vi "SMR_LabVIEW_V9.1.vi"() -> ()   [LabVIEW 2025]
uses:
  Control 1.ctl
  <vilib>/DAQmx/write.llb/DAQmx Write (Analog DBL 1Chan 1Samp).vi
  <vilib>/DAQmx/read.llb/DAQmx Read (Analog 1D DBL NChan 1Samp).vi
  <vilib>/DAQmx/read.llb/DAQmx Read (Analog 2D DBL NChan NSamp).vi
  <vilib>/Analysis/baseanly.llb/Mean (DBL).vi
  <vilib>/DAQmx/create/channels.llb/DAQmx Create Channel (AI-Temperature-Thermocouple).vi
  <vilib>/DAQmx/create/channels.llb/DAQmx Create Channel (AI-Voltage-Basic).vi
  <vilib>/DAQmx/create/channels.llb/DAQmx Create Channel (AO-Voltage-Basic).vi
  <vilib>/DAQmx/miscellaneous.llb/DAQmx Fill In Error Info.vi
  <vilib>/DAQmx/configure/timing.llb/DAQmx Timing (Sample Clock).vi
  <vilib>/DAQmx/create/channels.llb/DAQmx Create Channel (AO-Current-Basic).vi
  <vilib>/addons/control/pid/pid.llb/PID (DBL).vi
  <vilib>/measure/maspectr.llb/FFT Power Spectrum and PSD for 1 Chan.vi
  <vilib>/measure/matone.llb/Extract Single Tone Information 1 Chan.vi
  <vilib>/addons/control/pid/NI_PID_pid.lvlib
  <vilib>/Analysis/NI_AALBase.lvlib
  <vilib>/ptbypt/NI_PtbyPt.lvlib
  <vilib>/measure/NI_MAPro.lvlib
panel:
  in  "R Burden (Ohm)":T1=220.0 min=220.0 max=220.0
  out "PSU Command (mA)":dbl
  in  "PSU Power Setpoint (W)":dbl
  in  "Manual PSU Command (0-8.5)":dbl min=0.0 max=8.5
  in  "PSU: Manual/ PID (on)":bool
  out "Room Temp (deg C)":dbl
  out "HW Valve Command (V)":dbl
  in  "HX Flow Setpoint (GPM)":dbl
  in  "Manual HW Valve Command (V)":dbl min=0.0 max=10.0
  in  "HW Valve: Manual / PID (on)":bool
  in  "PID gains for HW Valve":T2={"proportional gain (Kc)"=1.0, "integral time (Ti, min)"=0.01, "derivative time (Td, min)"=0.0} {"derivative time (Td, min)" format="%.3f"; "integral time (Ti, min)" format="%.3f"; "proportional gain (Kc)" format="%.3f"}
  out "Rod Power (W)":dbl
  out "Current Through Rod (A)":dbl
  out "Time in Steady State (s)":dbl
  in  "Steady-State Dwell (s)":dbl
  out "Main Loop Flow (GPM)":dbl
  out "FM Amplitude":dbl
  out "FM Frequency":dbl
  out "Spectrum":cluster{"f0":dbl, "df":dbl, "magnitude":dbl[]}(graph)
  out "Raw Signal":waveform(dbl)(graph)
  out "Smoothed HX Flow (GPM)":dbl
  out "Flow History":dbl(graph)
  out "HX Flow (GPM)":dbl
  out "Voltage Across Rod (V)":dbl format="%0.2f"
  out "Current Run Folder":path
  in  "Log Root Folder":path=path "C:/Users/LocalUser/Documents/GitHub/thermal-loop/resources/v0.1.1/data/001"
  out "Raw NI9201 \nVoltage Display":T3
  in  "Loop Period (ms)":dbl=1000.0
  in  "Stop":bool
  out "Auto Steady State Threshold (deg C/min)":dbl
  out "Max dT/dt (deg C/min)":dbl
  out "Temp Change Rate (deg C/min)":dbl
  out "5-Min Baseline Complete":bool
  out "Rate Window Ready":bool
  out "Steady State":bool
  in  "Voltage Limit (V)":dbl=10.0
  in  "Temperature Limit (C)":dbl=50.0
  in  "Pressure Limit (psi)":dbl=15.0
  out "Max Voltage":bool
  out "Max Temperature":bool
  out "Max Pressure":bool
  out "Heat Exchanger Pressure History":dbl(graph)
  out "Main Loop Pressure History":T4(graph)
  out "Overall Avg Pressure (psi)":dbl
  out "Heat Exchanger Pressure P6 (psi)":dbl
  out "Main Loop Avg Pressure (psi)":dbl
  out "Pressure Display":T5
  out "Overall Pressure History":T6(graph)
  out "Max Loop Pressure (psi)":dbl
  out "Heat Exchanger Temperature History":cluster{"Waveform":dbl, "Waveform":dbl}(graph)
  out "Main Loop Temeperature History":T7(graph)
  out "Heat Exchanger Avg Temp (deg C)":dbl
  out "Temperature Display":T8
  out "Overall Temperature History":T9(graph)
  out "Overall Avg Temp (deg C)":dbl
  out "Max Loop Temp (deg C)":dbl
  out "Final P-Valve Voltage (V)":dbl
  out "PID Trim Voltage (V)":dbl
  in  "PID Temp Setpoint (deg C)":dbl
  in  "Auto PID Enable":bool
  in  "Manual P-Valve Voltage (V)":dbl min=0.0 max=10.0
  out "Main Loop Avg Temp (deg C)":dbl
  # "PSU Control"
  # "HoneyWell Valve Control"
  # "Heat Exchanger Flow"
  # "Control/Troubleshoot"
  # "Steady State"
  # "Emergency Indicators"
  # "Pressure"
  # "Temperature"
  # "Proportional Valve Control"
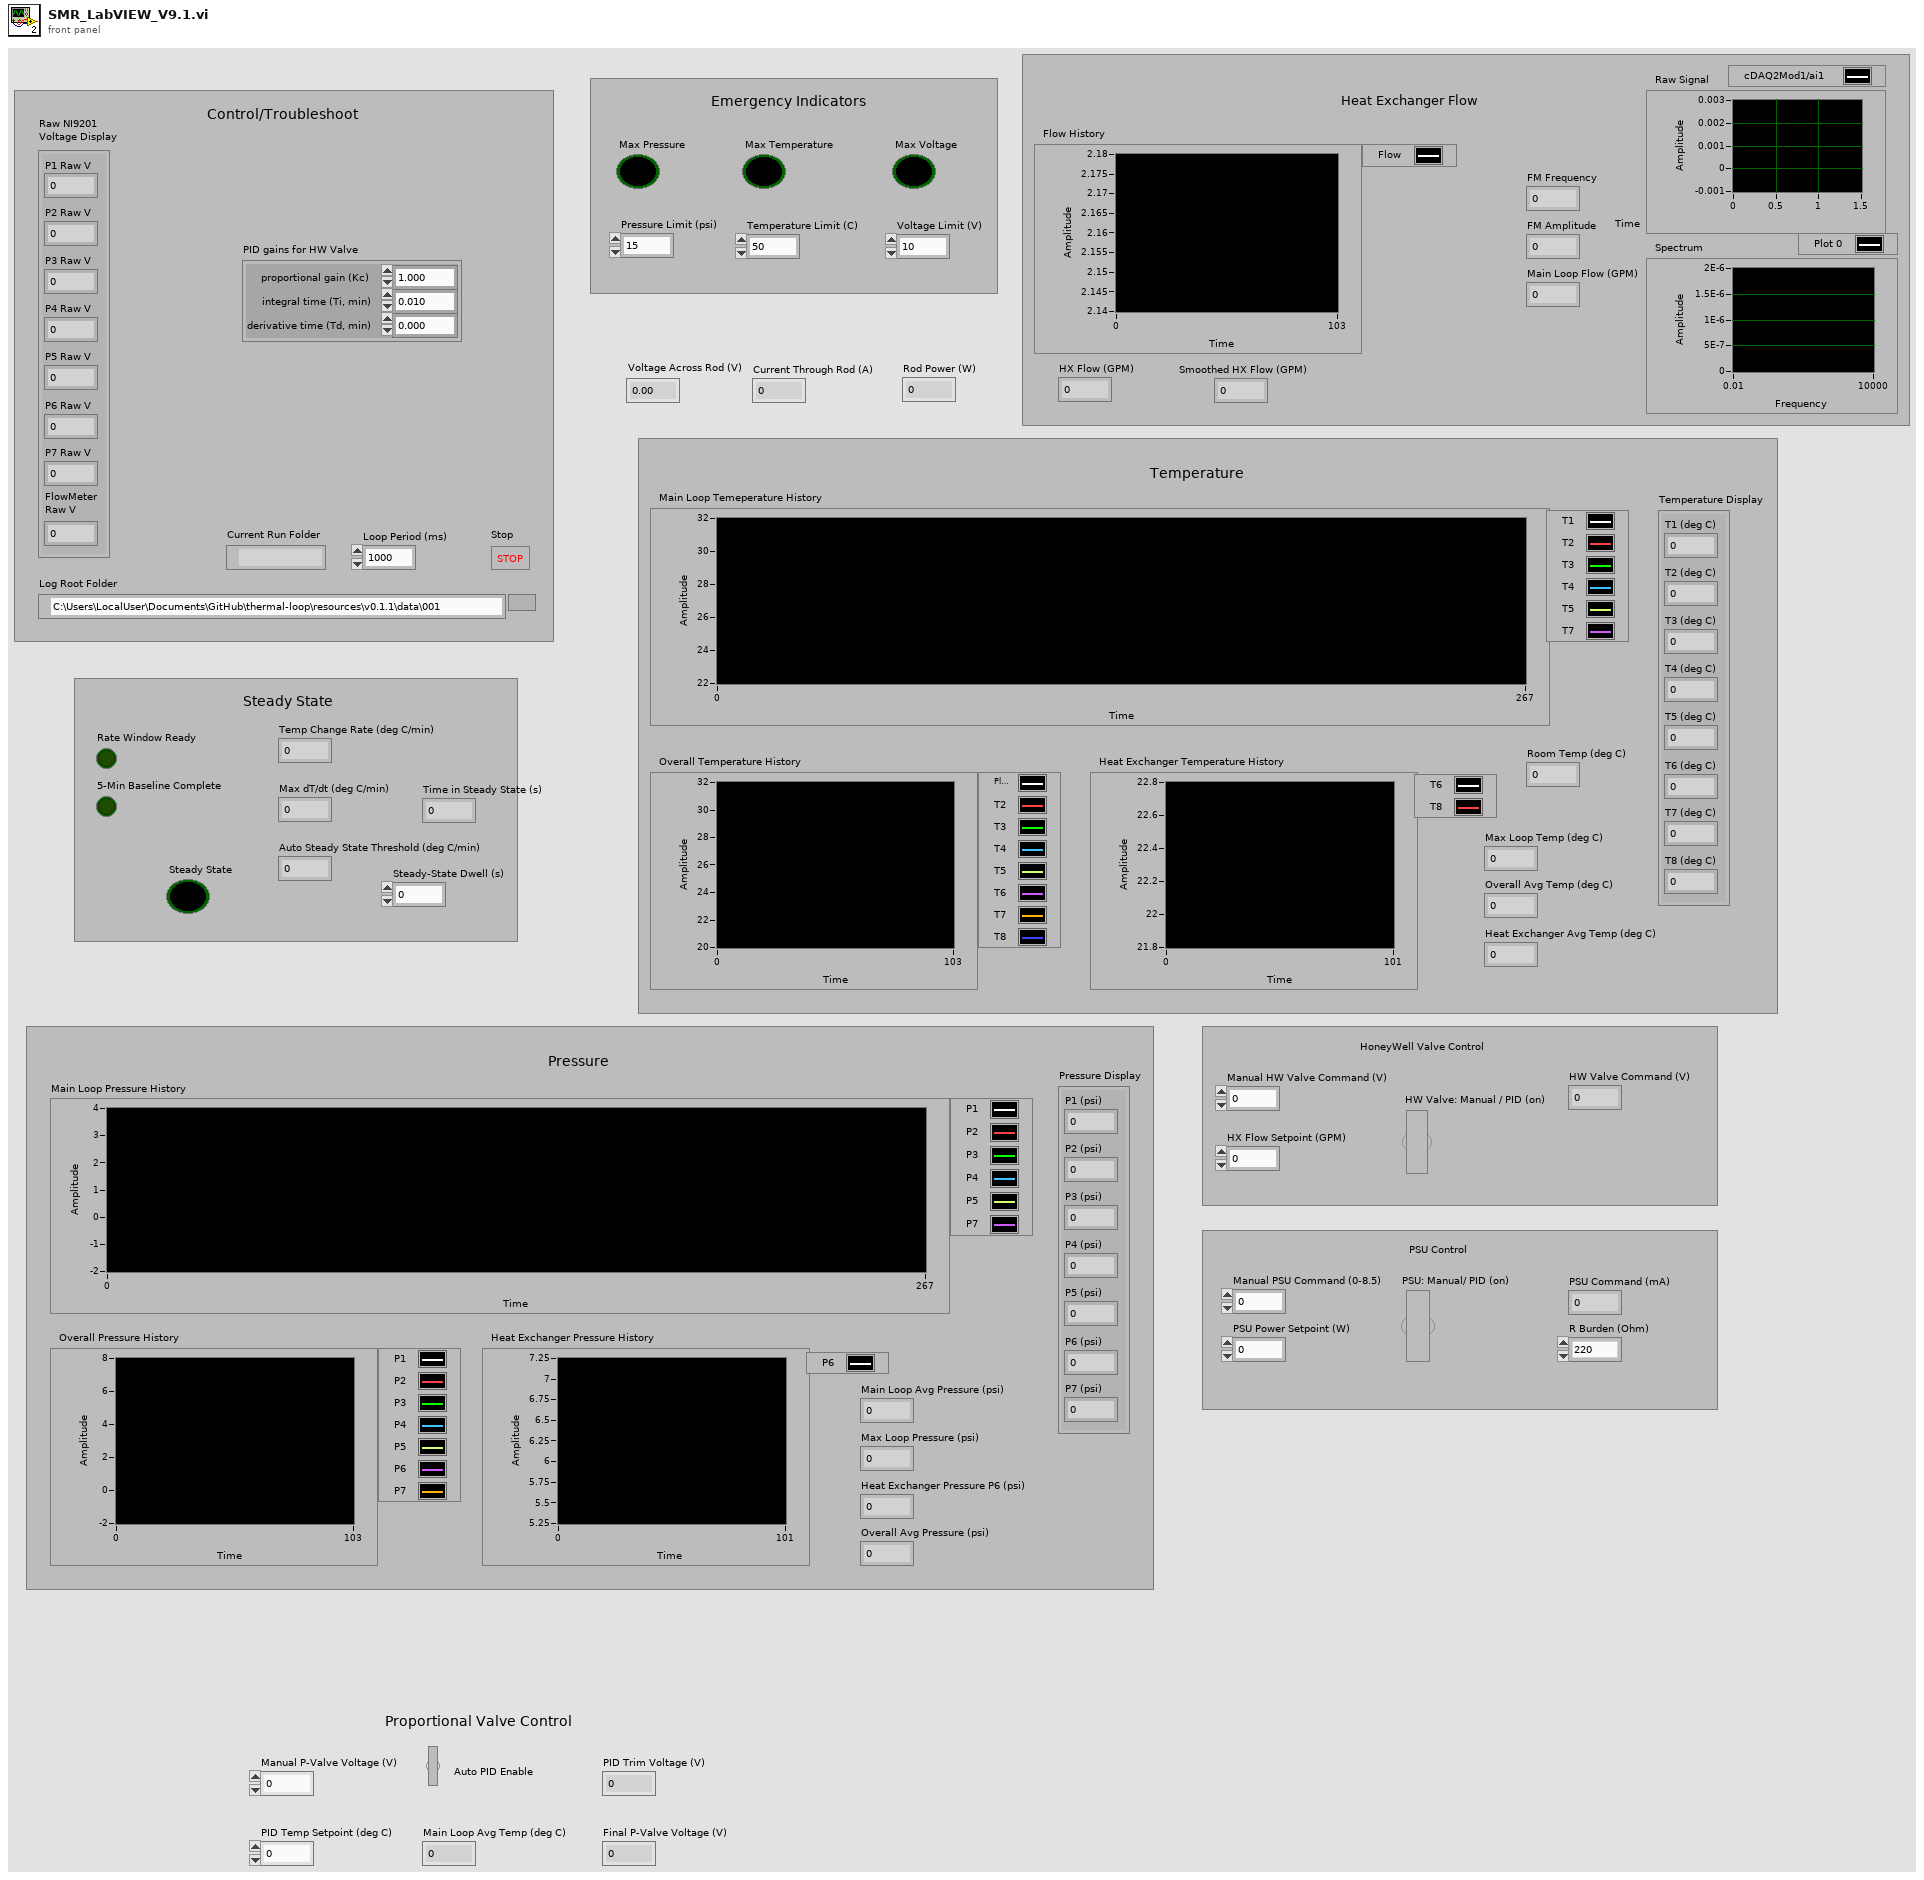
[diagram p1: front panel]
types:
  T1 = typedef "Control 1.ctl" = dbl
  T2 = cluster{"proportional gain (Kc)":dbl, "integral time (Ti, min)":dbl, "derivative time (Td, min)":dbl}
  T3 = cluster{"P1 Raw V":dbl, "P2 Raw V":dbl, "P3 Raw V":dbl, "P4 Raw V":dbl, "P5 Raw V":dbl, "P6 Raw V":dbl, "P7 Raw V":dbl, "FlowMeter\nRaw V":dbl}
  T4 = cluster{"P1":dbl, "P2":dbl, "P3":dbl, "P4":dbl, "P5":dbl, "P7":dbl}
  T5 = cluster{"P1 (psi)":dbl, "P2 (psi)":dbl, "P3 (psi)":dbl, "P4 (psi)":dbl, "P5 (psi)":dbl, "P6 (psi)":dbl, "P7 (psi)":dbl}
  T6 = cluster{"P1":dbl, "P2":dbl, "P3":dbl, "P4":dbl, "P5":dbl, "P6":dbl, "P7":dbl}
  T7 = cluster{"Waveform":dbl, "Waveform":dbl, "Waveform":dbl, "Waveform":dbl, "Waveform":dbl, "Waveform":dbl}
  T8 = cluster{"T1 (deg C)":dbl, "T2 (deg C)":dbl, "T3 (deg C)":dbl, "T4 (deg C)":dbl, "T5 (deg C)":dbl, "T6 (deg C)":dbl, "T7 (deg C)":dbl, "T8 (deg C)":dbl}
  T9 = cluster{"Waveform":dbl, "Waveform":dbl, "Waveform":dbl, "Waveform":dbl, "Waveform":dbl, "Waveform":dbl, "Waveform":dbl, "Waveform":dbl}
  T10 = enum16{"open", "replace", "create", "open or create", "replace or create", "replace or create with confirmation"}
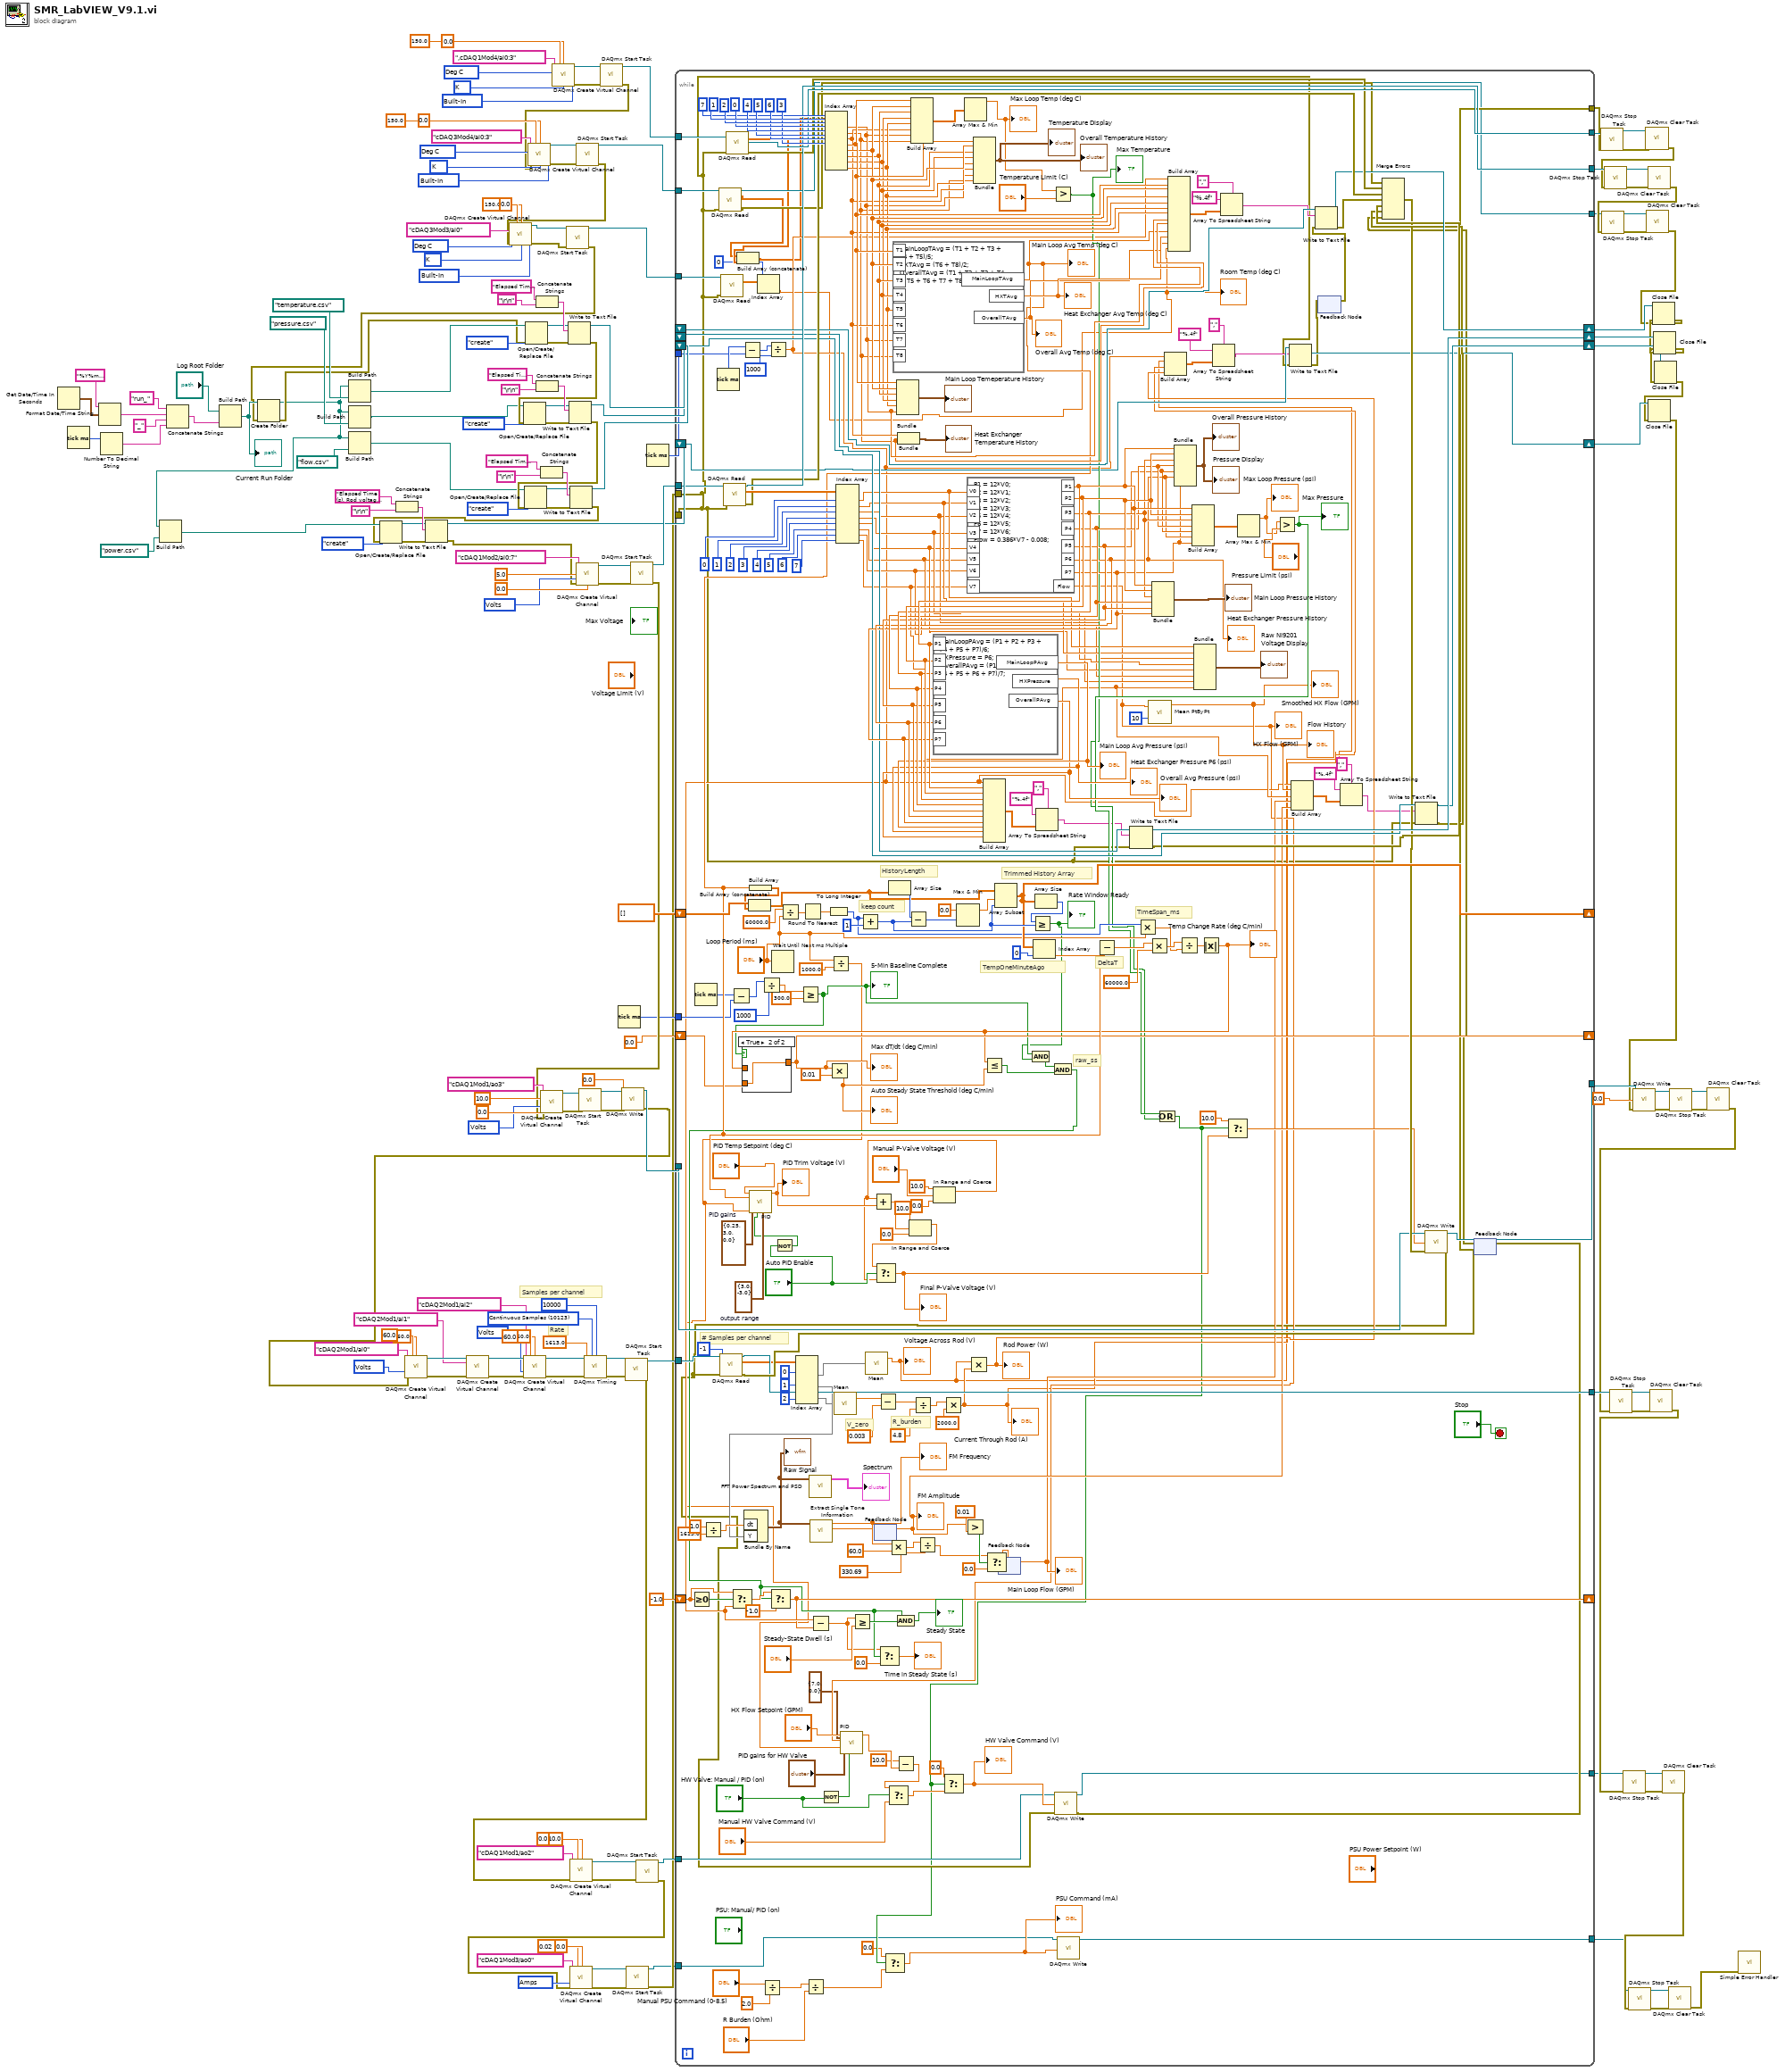
[diagram p0: block diagram]
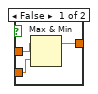
[diagram p2: hidden frame]
diagram:
  w9 = 10342 items=["Amps"=10342, "From Custom Scale"=10065] ("units")
  w15 = 10200 items=["Built-In"=10200, "Constant Value"=10116, "Channel"=10113] ("cjc source")
  w16 = 10073 items=["J"=10072, "K"=10073, "N"=10077, "R"=10082, "S"=10085, "T"=10086, "B"=10047, "E"=10055] ("thermocouple type")
  w22 = 10143 items=["Deg C"=10143, "Deg F"=10144, "Kelvins"=10325, "Deg R"=10145, "From Custom Scale"=10065] ("units")
  w40 = 10348 items=["Volts"=10348, "From Custom Scale"=10065] ("units")
  w56 = 10200 items=["Built-In"=10200, "Constant Value"=10116, "Channel"=10113] ("cjc source")
  w57 = 10073 items=["J"=10072, "K"=10073, "N"=10077, "R"=10082, "S"=10085, "T"=10086, "B"=10047, "E"=10055] ("thermocouple type")
  w58 = 10143 items=["Deg C"=10143, "Deg F"=10144, "Kelvins"=10325, "Deg R"=10145, "From Custom Scale"=10065] ("units")
  w88 = 10123 items=["Finite Samples"=10178, "Continuous Samples"=10123, "Hardware Timed Single Point"=12522] ("sample mode")
  w90 = 10348 items=["Volts"=10348, "From Custom Scale"=10065] ("units")
  w109 = 10348 items=["Volts"=10348, "From Custom Scale"=10065] ("units")
  w171 = 10200 items=["Built-In"=10200, "Constant Value"=10116, "Channel"=10113] ("cjc source")
  w172 = 10073 items=["J"=10072, "K"=10073, "N"=10077, "R"=10082, "S"=10085, "T"=10086, "B"=10047, "E"=10055] ("thermocouple type")
  w173 = 10143 items=["Deg C"=10143, "Deg F"=10144, "Kelvins"=10325, "Deg R"=10145, "From Custom Scale"=10065] ("units")
  w180 = 10348 items=["Volts"=10348, "From Custom Scale"=10065] ("units")
  # "Samples per channel"
  # "Rate"
  n1 = Get Date/Time In Seconds() -> (seconds since 1Jan1904=w130:timestamp)
  n2 = Tick Count (ms)() -> (millisecond timer value=w128:u32)
  n3 = Format Date/Time String(time format string (%c)="%Y%m%d_%H%M%S", seconds (now)=w130) -> (date/time string=w125:string)  [unwired: 1 in]
  n4 = Number To Decimal String(number=w128) -> (decimal integer string=w126:string)  [unwired: 1 in]
  n5 = Concatenate Strings("run_" ("string"), w125, "_" ("string"), w126) -> (w122:string)
  n6 = Build Path(base path="Log Root Folder", name or relative path=w122) -> (appended path=w121:path)
  "Current Run Folder" <- w121
  n7 = Concatenate Strings("Elapsed Time (s), Rod voltage (V), Rod Current (A), Rod Power (W)", "\r\n") -> (w75:string)
  n8 = Concatenate Strings("Elapsed Time (s),T1 (deg C),T2 (deg C),T3 (deg C),T4 (deg C),T5 (deg C),T6 (deg C),T7 (deg C),T8 (deg C),Main Loop Avg Temp (deg C),HX Avg Temp (deg C),Overall Avg Temp (deg C), Room Temp (deg C)", "\r\n") -> (w154:string)
  n9 = Concatenate Strings("Elapsed Time (s),P1 (psi),P2 (psi),P3 (psi),P4 (psi),P5 (psi),P6 (psi),P7 (psi),Main Loop Avg Pressure (psi),HX Pressure (psi),Overall Avg Pressure (psi)", "\r\n") -> (w152:string)
  n10 = Concatenate Strings("Elapsed Time (s),Heat Exchanger Flow (GPM),Flow Raw Voltage (V), Main Loop Flow (GPM), Flow Signal Amplitude (V)", "\r\n") -> (w148:string)
  n11 = call-poly <vilib>:"DAQmx Create Virtual Channel.vi"("maximum value"=150.0, "minimum value"=0.0, "physical channels"=tag ",cDAQ1Mod4/ai0:3", "cjc source"=w171, "units"=w173, "thermocouple type"=w172) -> ("task out"=w170:refnum<k21>, "error out"=w169:errorcluster)  [unwired: 8 in]
  n12 = call <vilib>:"DAQmx Start Task.vi"("task/channels in"=w170, "error in"=w169) -> ("task out"=w168:refnum<k21>, "error out"=w52:errorcluster)  [unwired: 12 in]
  n13 = call-poly <vilib>:"DAQmx Create Virtual Channel.vi"("maximum value"=150.0, "minimum value"=0.0, "physical channels"=tag "cDAQ3Mod4/ai0:3", "cjc source"=w56, "units"=w58, "error in"=w52, "thermocouple type"=w57) -> ("task out"=w55:refnum<k21>, "error out"=w54:errorcluster)  [unwired: 7 in]
  n14 = call <vilib>:"DAQmx Start Task.vi"("task/channels in"=w55, "error in"=w54) -> ("task out"=w51:refnum<k21>, "error out"=w19:errorcluster)  [unwired: 12 in]
  n15 = call-poly <vilib>:"DAQmx Create Virtual Channel.vi"("maximum value"=150.0, "minimum value"=0.0, "physical channels"=tag "cDAQ3Mod3/ai0", "cjc source"=w15, "units"=w22, "error in"=w19, "thermocouple type"=w16) -> ("task out"=w21:refnum<k21>, "error out"=w20:errorcluster)  [unwired: 7 in]
  n16 = call <vilib>:"DAQmx Start Task.vi"("task/channels in"=w21, "error in"=w20) -> ("task out"=w17:refnum<k21>, "error out"=w18:errorcluster)  [unwired: 12 in]
  n17 = Create Folder(path (use dialog)=w121, error in=w18) -> (created path=w69:path, error out=w114:errorcluster)  [unwired: 1 in, 1 out]
  n18 = Build Path(base path=w69, name or relative path=path "power.csv") -> (appended path=w70:path)
  n19 = Build Path(base path=w69, name or relative path=path "temperature.csv") -> (appended path=w120:path)
  n20 = Build Path(base path=w69, name or relative path=path "pressure.csv") -> (appended path=w119:path)
  n21 = Build Path(base path=w69, name or relative path=path "flow.csv") -> (appended path=w118:path)
  n22 = Open/Create/Replace File(file path (use dialog)=w120, error in=w114, operation (0:open)=T10."create") -> (refnum out=w153:refnum<file>, error out=w137:errorcluster)  [unwired: 3 in, 1 out]
  n23 = Write to Text File(file (use dialog)=w153, text=w154, error in=w137) -> (refnum out=w144:refnum<file>, error out=w136:errorcluster)  [unwired: 1 in, 1 out]
  n24 = Open/Create/Replace File(file path (use dialog)=w119, error in=w136, operation (0:open)=T10."create") -> (refnum out=w151:refnum<file>, error out=w135:errorcluster)  [unwired: 3 in, 1 out]
  n25 = Write to Text File(file (use dialog)=w151, text=w152, error in=w135) -> (refnum out=w143:refnum<file>, error out=w134:errorcluster)  [unwired: 1 in, 1 out]
  n26 = Open/Create/Replace File(file path (use dialog)=w118, error in=w134, operation (0:open)=T10."create") -> (refnum out=w147:refnum<file>, error out=w133:errorcluster)  [unwired: 3 in, 1 out]
  n27 = Write to Text File(file (use dialog)=w147, text=w148, error in=w133) -> (refnum out=w142:refnum<file>, error out=w67:errorcluster)  [unwired: 1 in, 1 out]
  n28 = Open/Create/Replace File(file path (use dialog)=w70, error in=w67, operation (0:open)=T10."create") -> (refnum out=w74:refnum<file>, error out=w71:errorcluster)  [unwired: 3 in, 1 out]
  n29 = Write to Text File(file (use dialog)=w74, text=w75, error in=w71) -> (refnum out=w65:refnum<file>, error out=w66:errorcluster)  [unwired: 1 in, 1 out]
  n30 = call-poly <vilib>:"DAQmx Create Virtual Channel.vi"("maximum value"=5.0, "minimum value"=0.0, "physical channels"=tag "cDAQ1Mod2/ai0:7", "units"=w180, "error in"=w66) -> ("task out"=w179:refnum<k21>, "error out"=w178:errorcluster)  [unwired: 9 in]
  n31 = Tick Count (ms)() -> (millisecond timer value=w95:u32)
  n32 = call <vilib>:"DAQmx Start Task.vi"("task/channels in"=w179, "error in"=w178) -> ("task out"=w177:refnum<k21>, "error out"=w102:errorcluster)  [unwired: 12 in]
  n33 = call-poly <vilib>:"DAQmx Create Virtual Channel.vi"("maximum value"=10.0, "minimum value"=0.0, "physical channels"=tag "cDAQ1Mod1/ao3", "units"=w109, "error in"=w102) -> ("task out"=w108:refnum<k21>, "error out"=w107:errorcluster)  [unwired: 9 in]
  n34 = call <vilib>:"DAQmx Start Task.vi"("task/channels in"=w108, "error in"=w107) -> ("task out"=w106:refnum<k21>, "error out"=w105:errorcluster)  [unwired: 12 in]
  n35 = call-poly <vilib>:"DAQmx Write.vi"("task/channels in"=w106, "data"=0.0, "error in"=w105) -> ("task out"=w103:refnum<k21>, "error out"=w82:errorcluster)  [unwired: 10 in, 1 out]
  n36 = call-poly <vilib>:"DAQmx Create Virtual Channel.vi"("maximum value"=60.0, "minimum value"=-60.0, "physical channels"=tag "cDAQ2Mod1/ai0", "units"=w90, "error in"=w82) -> ("task out"=w79:refnum<k21>, "error out"=w78:errorcluster)  [unwired: 9 in]
  n37 = call-poly <vilib>:"DAQmx Create Virtual Channel.vi"("task in"=w79, "physical channels"=tag "cDAQ2Mod1/ai1", "error in"=w78) -> ("task out"=w44:refnum<k21>, "error out"=w42:errorcluster)  [unwired: 11 in]
  n38 = call-poly <vilib>:"DAQmx Create Virtual Channel.vi"("task in"=w44, "maximum value"=60.0, "minimum value"=-60.0, "physical channels"=tag "cDAQ2Mod1/ai2", "units"=w40, "error in"=w42) -> ("task out"=w43:refnum<k21>, "error out"=w41:errorcluster)  [unwired: 8 in]
  n39 = call-poly <vilib>:"DAQmx Timing.vi"("task/channels in"=w43, "sample mode"=w88, "samples per channel"=10000, "rate"=1613.0, "error in"=w41) -> ("task out"=w86:refnum<k21>, "error out"=w85:errorcluster)  [unwired: 9 in]
  n40 = call <vilib>:"DAQmx Start Task.vi"("task/channels in"=w86, "error in"=w85) -> ("task out"=w81:refnum<k21>, "error out"=w31:errorcluster)  [unwired: 12 in]
  n41 = call-poly <vilib>:"DAQmx Create Virtual Channel.vi"("maximum value"=10.0, "minimum value"=0.0, "physical channels"=tag "cDAQ1Mod1/ao2", "error in"=w31) -> ("task out"=w34:refnum<k21>, "error out"=w33:errorcluster)  [unwired: 10 in]
  n42 = call <vilib>:"DAQmx Start Task.vi"("task/channels in"=w34, "error in"=w33) -> ("task out"=w32:refnum<k21>, "error out"=w8:errorcluster)  [unwired: 12 in]
  n43 = call-poly <vilib>:"DAQmx Create Virtual Channel.vi"("maximum value"=0.02, "minimum value"=0.0, "physical channels"=tag "cDAQ1Mod3/ao0", "units"=w9, "error in"=w8) -> ("task out"=w14:refnum<k21>, "error out"=w13:errorcluster)  [unwired: 9 in]
  n44 = call <vilib>:"DAQmx Start Task.vi"("task/channels in"=w14, "error in"=w13) -> ("task out"=w1:refnum<k21>, "error out"=w7:errorcluster)  [unwired: 12 in]
  n45 = Tick Count (ms)() -> (millisecond timer value=w141:u32)
  n46 = while {
    tunnel: w177 -> [w432]
    tunnel: w168 -> [w415]
    tunnel: [w406] -> w167
    tunnel: [w197] -> _
    tunnel: [w405] -> w166
    tunnel: [w293] -> w165
    shift-right: [w384] -> w140
    shift-left: w144 -> [w385]
    shift-right: [w369] -> w139
    shift-left: w143 -> [w370]
    shift-right: [w364] -> w138
    shift-left: w142 -> [w365]
    tunnel: w141 -> [w401]
    shift-right: [w343] -> _
    shift-left: dbl[] [] -> [w356]
    tunnel: w103 -> [w325]
    tunnel: w7 -> [w197]
    tunnel: [w331] -> w100
    tunnel: w95 -> [w314]
    shift-right: [w307] -> _
    shift-left: 0.0 -> [w309]
    tunnel: w81 -> [w292]
    tunnel: [w291] -> w80
    shift-right: [w254] -> w64
    shift-left: w65 -> [w255]
    shift-right: [w246] -> _
    shift-left: -1.0 -> [w250]
    tunnel: w51 -> [w238]
    tunnel: [w236] -> w47
    tunnel: w32 -> [w216]
    tunnel: [w212] -> w26
    tunnel: w17 -> [w198]
    tunnel: [w185] -> w2
    tunnel: w1 -> [w184]
    stop <- "Stop" stop-if-true
    w329 = cluster{"output high":dbl, "output low":dbl} {"output high"=3.0, "output low"=-3.0}  # output range
    w330 = T2 {"proportional gain (Kc)"=0.25, "integral time (Ti, min)"=3.0, "derivative time (Td, min)"=0.0}  # PID gains
    # "R_burden"
    # "V_zero"
    # "raw_ss"
    # "# Samples per channel"
    # "TimeSpan_ms"
    # "DeltaT"
    # "TempOneMinuteAgo"
    # "Trimmed History Array"
    # "HistoryLength"
    # "keep count"
    n47 = Greater Or Equal To 0?(x=w250) -> (x >= 0?=w251:bool)
    n48 = Tick Count (ms)() -> (millisecond timer value=w315:u32)
    n49 = Divide(x=1.0, y=1613.0) -> (x/y=w265:dbl)
    n50 = Tick Count (ms)() -> (millisecond timer value=w402:u32)
    n51 = call-poly <vilib>:"DAQmx Read.vi"("task/channels in"=w238, "error in"=w197) -> ("task out"=w236:refnum<k21>, "data"=w233:dbl[], "error out"=w237:errorcluster)  [unwired: 11 in]
    n52 = call-poly <vilib>:"DAQmx Read.vi"("task/channels in"=w198, "error in"=w197) -> ("data"=w195:dbl[])  [unwired: 11 in, 2 out]
    n53 = call-poly <vilib>:"DAQmx Read.vi"("task/channels in"=w432, "error in"=w197) -> ("task out"=w405:refnum<k21>, "data"=w423:dbl[], "error out"=w403:errorcluster)  [unwired: 11 in]
    n54 = call-poly <vilib>:"DAQmx Read.vi"("task/channels in"=w415, "error in"=w197) -> ("task out"=w406:refnum<k21>, "data"=w234:dbl[], "error out"=w404:errorcluster)  [unwired: 11 in]
    n55 = Subtract(x=w315, y=w314) -> (x-y=w313:u32)
    n56 = Build Array (concatenate)(w233, w234) -> (w235:dbl[])
    n57 = Subtract(x=w402, y=w401) -> (x-y=w400:u32)
    n58 = Index Array(array=w195, index=0) -> (element=w194:dbl)
    "Room Temp (deg C)" <- w194
    n59 = Divide(x=w313, y=u32 1000) -> (x/y=w311:dbl)
    n60 = Divide(x="Manual PSU Command (0-8.5)", y=2.0) -> (x/y=w190:dbl)
    n61 = Divide(x=w400, y=u32 1000) -> (x/y=w247:dbl)
    n62 = Select(t=w250, s=w251, f=w247) -> (s? t:f=w249:dbl)
    n63 = Wait Until Next ms Multiple(millisecond multiple="Loop Period (ms)") -> ()  [unwired: 1 out]
    n64 = Not(x="Auto PID Enable") -> (.not. x?=w326:bool)
    n65 = Divide(x=60000.0, y="Loop Period (ms)") -> (x/y=w353:dbl)
    n66 = Greater Or Equal?(x=w311, y=300.0) -> (x >= y?=w304:bool)
    "5-Min Baseline Complete" <- w304
    n67 = Round To Nearest(number=w353) -> (nearest integer value=w352:dbl)
    n68 = Divide(x=w190, y="R Burden (Ohm)") -> (x/y=w187:T1)
    n69 = Not(x="HW Valve: Manual / PID (on)") -> (.not. x?=w225:bool)
    n70 = Index Array(array=w235, index #1=7 ("index"), index #2=1 ("index"), index #3=2 ("index"), index #4=0 ("index"), index #5=4 ("index"), index #6=5 ("index"), index #7=6 ("index"), index #8=3 ("index")) -> (element #1=w392:dbl, element #2=w391:dbl, element #3=w393:dbl, element #4=w398:dbl, element #5=w397:dbl, element #6=w396:dbl, element #7=w395:dbl, element #8=w394:dbl)
    n71 = To Long Integer(number=w352) -> (32bit integer=w340:i32)
    n72 = Divide(x="Loop Period (ms)", y=1000.0) -> (x/y=w211:dbl)
    n73 = Index Array(array=w423, index #1=0 ("index"), index #2=1 ("index"), index #3=2 ("index"), index #4=3 ("index"), index #5=4 ("index"), index #6=5 ("index"), index #7=6 ("index"), index #8=7 ("index")) -> (element #1=w290:dbl, element #2=w289:dbl, element #3=w288:dbl, element #4=w287:dbl, element #5=w286:dbl, element #6=w285:dbl, element #7=w284:dbl, element #8=w283:dbl)
    n74 = Add(x=w340, y=1) -> (x+y=w345:i32)
    n75 = feedback #1() -> (w261:dbl)  [unwired: 1 in]
    "FM Amplitude" <- w261
    n76 = formula code="MainLoopTAvg = (T1 + T2 + T3 + T4 + T5)/5;\nHXTAvg = (T6 + T8)/2;\nOverallTAvg = (T1 + T2 + T3 + T4 + T5 + T6 + T7 + T8)/8;"("T1"=w398, "T2"=w397, "T3"=w396, "T4"=w395, "T5"=w394, "T6"=w393, "T7"=w392, "T8"=w391) -> ("MainLoopTAvg"=w317:dbl, "HXTAvg"=w390:dbl, "OverallTAvg"=w389:dbl)
    "Overall Avg Temp (deg C)" <- w389
    "Main Loop Avg Temp (deg C)" <- w317
    "Heat Exchanger Avg Temp (deg C)" <- w390
    n77 = Build Array(w317) -> (w355:dbl[])
    n78 = Build Array (concatenate)(w356, w355) -> (w347:dbl[])
    n79 = call-poly <vilib>:"PID.vi"("reinitialize? (F)"=w326, "output range"=w329, "dt (s)"=w211, "PID gains"=w330, "process variable"=w317, "setpoint"="PID Temp Setpoint (deg C)") -> ("output"=w324:dbl)  [unwired: 4 in, 1 out]
    "PID Trim Voltage (V)" <- w324
    n80 = Array Size(array=w347) -> (size(s)=w350:i32)
    n81 = Bundle("Waveform"=w398, "Waveform"=w397, "Waveform"=w396, "Waveform"=w395, "Waveform"=w394, "Waveform"=w392) -> (→"Main Loop Temeperature History":T7)  [unwired: 1 in]
    n82 = Bundle("Waveform"=w393, "Waveform"=w391) -> (→"Heat Exchanger Temperature History":cluster{"Waveform":dbl, "Waveform":dbl})  [unwired: 1 in]
    n83 = Subtract(x=w350, y=w345) -> (x-y=w348:i32)
    n84 = Build Array(w398, w397, w396, w395, w394, w393, w392, w391) -> (w433:dbl[])
    n85 = In Range and Coerce(upper limit=10.0, x="Manual P-Valve Voltage (V)", lower limit=0.0) -> (coerced(x)=w319:dbl)  [unwired: 1 out]
    n86 = Add(x=w319, y=w324) -> (x+y=w323:dbl)
    n87 = In Range and Coerce(upper limit=10.0, x=w323, lower limit=0.0) -> (coerced(x)=w318:dbl)  [unwired: 1 out]
    n88 = Select(t=w318, s="Auto PID Enable", f=w319) -> (s? t:f=w296:dbl)
    "Final P-Valve Voltage (V)" <- w296
    n89 = Max & Min(x=0.0, y=w348) -> (max(x,y)=w346:dbl)  [unwired: 1 out]
    n90 = Array Max & Min(array=w433) -> (max value=w358:dbl)  [unwired: 3 out]
    "Max Loop Temp (deg C)" <- w358
    n91 = Greater?(x=w261, y=0.01) -> (0:w269:bool)
    n92 = formula code="P1 = 12*V0;\nP2 = 12*V1;\nP3 = 12*V2;\nP4 = 12*V3;\nP5 = 12*V4;\nP6 = 12*V5; \nP7 = 12*V6;\nFlow = 0.386*V7 - 0.008;"("V0"=w290, "V1"=w289, "V2"=w288, "V3"=w287, "V4"=w286, "V5"=w285, "V6"=w284, "V7"=w283) -> ("P1"=w383:dbl, "P2"=w382:dbl, "P3"=w381:dbl, "P4"=w380:dbl, "P5"=w379:dbl, "P6"=w378:dbl, "P7"=w377:dbl, "Flow"=w228:dbl)
    "HX Flow (GPM)" <- w228
    "Heat Exchanger Pressure History" <- w378
    n93 = call-poly <vilib>:"PID.vi"("reinitialize? (F)"=w225, "output range"=cluster{"output high":dbl, "output low":dbl} {"output high"=7.0, "output low"=0.0}, "dt (s)"=w211, "PID gains"="PID gains for HW Valve", "process variable"=w228, "setpoint"="HX Flow Setpoint (GPM)") -> ("output"=w224:dbl)  [unwired: 4 in, 1 out]
    n94 = Subtract(x=10.0, y=w224) -> (x-y=w221:dbl)
    n95 = Select(t=w221, s="HW Valve: Manual / PID (on)", f="Manual HW Valve Command (V)") -> (s? t:f=w219:dbl)
    n96 = formula code="MainLoopPAvg = (P1 + P2 + P3 + P4 + P5 + P7)/6;\nHXPressure = P6;\nOverallPAvg = (P1 + P2 + P3 + P4 + P5 + P6 + P7)/7;"("P1"=w383, "P2"=w382, "P3"=w381, "P4"=w380, "P5"=w379, "P6"=w378, "P7"=w377) -> ("MainLoopPAvg"=w376:dbl, "HXPressure"=w375:dbl, "OverallPAvg"=w374:dbl)
    "Overall Avg Pressure (psi)" <- w374
    "Heat Exchanger Pressure P6 (psi)" <- w375
    "Main Loop Avg Pressure (psi)" <- w376
    n97 = Bundle("Waveform"=w398, "Waveform"=w397, "Waveform"=w396, "Waveform"=w395, "Waveform"=w394, "Waveform"=w393, "Waveform"=w392, "Waveform"=w391) -> (→"Overall Temperature History" →"Temperature Display":T9)  [unwired: 1 in]
    n98 = Build Array(w247, w383, w382, w381, w380, w379, w378, w377, w376, w375, w374) -> (w373:dbl[])
    n99 = Array Subset(array=w347, index=w346, length=w345) -> (w343:dbl[])
    n100 = feedback #2() -> (w259:dbl)  [unwired: 1 in]
    "Main Loop Flow (GPM)" <- w259
    n101 = Index Array(array=w343, index=0) -> (element=w341:dbl)
    n102 = Array Size(array=w343) -> (size(s)=w344:i32)
    n103 = Greater Or Equal?(x=w344, y=w345) -> (x >= y?=w303:bool)
    "Rate Window Ready" <- w303
    n104 = And(x=w304, y=w303) -> (x .and. y?=w302:bool)
    n105 = Array To Spreadsheet String(delimiter (Tab)=",", array=w373, 3:"%.4f" ("format string")) -> (spreadsheet string=w207:string)
    n106 = Greater?(x=w358, y="Temperature Limit (C)") -> (0:w299:bool)
    "Max Temperature" <- w299
    n107 = Subtract(x=w317, y=w341) -> (x-y=w339:dbl)
    n108 = Write to Text File(file (use dialog)=w370, text=w207, error in=w197) -> (refnum out=w369:refnum<file>, error out=w362:errorcluster)  [unwired: 1 in, 1 out]
    n109 = Multiply(x=w340, y="Loop Period (ms)") -> (x*y=w336:dbl)
    n110 = Multiply(x=w339, y=60000.0) -> (x*y=w337:dbl)
    n111 = call <vilib>:"Mean PtByPt.vi"("x"=w228, "sample length"=10) -> ("mean"=w281:dbl)  [unwired: 2 in, 1 out]
    "Flow History" <- w281
    "Smoothed HX Flow (GPM)" <- w281
    n112 = Bundle("P1"=w383, "P2"=w382, "P3"=w381, "P4"=w380, "P5"=w379, "P7"=w377) -> (→"Main Loop Pressure History":T4)  [unwired: 1 in]
    n113 = Build Array(w247, w398, w397, w396, w395, w394, w393, w392, w391, w317, w390, w389, w194) -> (w388:dbl[])
    n114 = Bundle("P1"=w383, "P2"=w382, "P3"=w381, "P4"=w380, "P5"=w379, "P6"=w378, "P7"=w377) -> (→"Overall Pressure History" →"Pressure Display":T6)  [unwired: 1 in]
    n115 = Divide(x=w337, y=w336) -> (x/y=w335:dbl)
    n116 = Build Array(w383, w382, w381, w380, w379, w378, w377) -> (w422:dbl[])
    n117 = Bundle("Waveform"=w290, "Waveform"=w289, "Waveform"=w288, "Waveform"=w287, "Waveform"=w286, "Waveform"=w285, "Waveform"=w284, "Waveform"=w283) -> (→"Raw NI9201 \nVoltage Display":T9)  [unwired: 1 in]
    n118 = Absolute Value(x=w335) -> (abs(x)=w306:dbl)
    "Temp Change Rate (deg C/min)" <- w306
    n119 = case shown="True" w304 {
      tunnel: w309 -> [w437 w438]
      tunnel: w306 -> [w436 _]
      tunnel: [w435 w438] -> w307
      frame False {
        n120 = Max & Min(x=w436, y=w437) -> (max(x,y)=w435:dbl)  [unwired: 1 out]
      }
      frame True {
      }
    }
    "Max dT/dt (deg C/min)" <- w307
    n121 = Multiply(x=w307, y=0.01) -> (x*y=w305:dbl)
    "Auto Steady State Threshold (deg C/min)" <- w305
    n122 = Less Or Equal?(x=w306, y=w305) -> (x <= y?=w301:bool)
    n123 = And(x=w302, y=w301) -> (x .and. y?=w242:bool)
    n124 = Select(t=w249, s=w242, f=-1.0) -> (s? t:f=w246:dbl)
    n125 = Subtract(x=w247, y=w246) -> (x-y=w241:dbl)
    n126 = Greater Or Equal?(x=w241, y="Steady-State Dwell (s)") -> (x >= y?=w244:bool)
    n127 = Select(t=w241, s=w242, f=0.0) -> (s? t:f=→"Time in Steady State (s)":dbl)
    n128 = And(x=w242, y=w244) -> (x .and. y?=→"Steady State":bool)
    n129 = Array To Spreadsheet String(delimiter (Tab)=",", array=w388, 3:"%.4f" ("format string")) -> (spreadsheet string=w208:string)
    n130 = Array Max & Min(array=w422) -> (max value=w359:dbl)  [unwired: 3 out]
    "Max Loop Pressure (psi)" <- w359
    n131 = Greater?(x=w359, y="Pressure Limit (psi)") -> (0:w300:bool)
    "Max Pressure" <- w300
    n132 = Or(x=w300, y=w299) -> (x .or. y?=w188:bool)
    n133 = Select(t=0.0, s=w188, f=w187) -> (s? t:f=w193:T1)
    "PSU Command (mA)" <- w193
    n134 = Select(t=0.0, s=w188, f=w219) -> (s? t:f=w217:dbl)
    "HW Valve Command (V)" <- w217
    n135 = call-poly <vilib>:"DAQmx Write.vi"("task/channels in"=w184, "data"=w193) -> ("task out"=w185:refnum<k21>)  [unwired: 11 in, 2 out]
    n136 = Select(t=10.0, s=w188, f=w296) -> (s? t:f=w295:dbl)
    n137 = Build Array(w247, w281, w283, w259, w261) -> (w368:dbl[])
    n138 = feedback #3() -> (w252:errorcluster)  [unwired: 1 in]
    n139 = Write to Text File(file (use dialog)=w385, text=w208, error in=w252) -> (refnum out=w384:refnum<file>, error out=w363:errorcluster)  [unwired: 1 in, 1 out]
    n140 = Array To Spreadsheet String(delimiter (Tab)=",", array=w368, 3:"%.4f" ("format string")) -> (spreadsheet string=w210:string)
    n141 = Write to Text File(file (use dialog)=w365, text=w210, error in=w197) -> (refnum out=w364:refnum<file>, error out=w361:errorcluster)  [unwired: 1 in, 1 out]
    n142 = feedback #4() -> (w213:errorcluster)  [unwired: 1 in]
    n143 = Merge Errors(w237, w404, w403, w363, w362, w361, w213) -> (w332:errorcluster)
    n144 = call-poly <vilib>:"DAQmx Write.vi"("task/channels in"=w325, "data"=w295, "error in"=w332) -> ("task out"=w331:refnum<k21>, "error out"=w215:errorcluster)  [unwired: 10 in, 1 out]
    n145 = call-poly <vilib>:"DAQmx Read.vi"("task/channels in"=w292, "number of samples per channel"=-1, "error in"=w215) -> ("task out"=w291:refnum<k21>, "data"=w280:dbl[][], "error out"=w293:errorcluster)  [unwired: 10 in]
    n146 = Index Array(array=w280, index (row) #1=0 ("index (row)"), index (row) #2=1 ("index (row)"), index (row) #3=2 ("index (row)")) -> (element #1=w279:dbl[], element #2=w264:dbl[], element #3=w231:dbl[])  [unwired: 3 in]
    n147 = Bundle By Name("dt"=w265, "Y"=w264) -> (w263:waveform(dbl))  [unwired: 1 in]
    "Raw Signal" <- w263
    n148 = call-poly <vilib>:"FFT Power Spectrum and PSD.vi"("time signal"=w263) -> ("Power Spectrum / PSD"=→"Spectrum":cluster{"f0":dbl, "df":dbl, "magnitude":dbl[]})  [unwired: 7 in, 3 out]
    n149 = call-poly <vilib>:"Extract Single Tone Information.vi"("time signal in"=w263) -> ("detected amplitude"=w262:dbl, "detected frequency"=w275:dbl)  [unwired: 5 in, 4 out]
    "FM Frequency" <- w275
    n150 = call-poly <vilib>:"Mean.vi"("X"=w231) -> ("mean"=w206:dbl)  [unwired: 1 out]
    n151 = call-poly <vilib>:"Mean.vi"("X"=w279) -> ("mean"=w199:dbl)  [unwired: 1 out]
    "Voltage Across Rod (V)" <- w199
    n152 = feedback-in #1(w262) -> ()
    n153 = Subtract(x=w206, y=0.003) -> (x-y=w204:dbl)
    n154 = Multiply(x=w275, y=60.0) -> (x*y=w273:dbl)
    n155 = Divide(x=w204, y=4.8) -> (x/y=w202:dbl)
    n156 = Divide(x=w273, y=330.69) -> (x/y=w268:dbl)
    n157 = Multiply(x=w202, y=2000.0) -> (x*y=w200:dbl)
    "Current Through Rod (A)" <- w200
    n158 = Multiply(x=w199, y=w200) -> (x*y=w230:dbl)
    "Rod Power (W)" <- w230
    n159 = Select(t=w268, s=w269, f=0.0) -> (s? t:f=w260:dbl)
    n160 = feedback-in #2(w260) -> ()
    n161 = call-poly <vilib>:"DAQmx Write.vi"("task/channels in"=w216, "data"=w217, "error in"=w215) -> ("task out"=w212:refnum<k21>, "error out"=w214:errorcluster)  [unwired: 10 in, 1 out]
    n162 = Build Array(w247, w199, w200, w230) -> (w256:dbl[])
    n163 = Array To Spreadsheet String(delimiter (Tab)=",", array=w256, 3:"%.4f" ("format string")) -> (spreadsheet string=w209:string)
    n164 = Write to Text File(file (use dialog)=w255, text=w209, error in=w197) -> (refnum out=w254:refnum<file>, error out=w253:errorcluster)  [unwired: 1 in, 1 out]
    n165 = feedback-in #3(w253) -> ()
    n166 = feedback-in #4(w214) -> ()
  }
  n167 = call <vilib>:"DAQmx Stop Task.vi"("task/channels in"=w167, "error in"=w165) -> ("task out"=w164:refnum<k21>, "error out"=w162:errorcluster)  [unwired: 12 in]
  n168 = call <vilib>:"DAQmx Clear Task.vi"("task in"=w164, "error in"=w162) -> ("error out"=w161:errorcluster)  [unwired: 13 in]
  n169 = call <vilib>:"DAQmx Stop Task.vi"("task/channels in"=w166, "error in"=w161) -> ("task out"=w163:refnum<k21>, "error out"=w160:errorcluster)  [unwired: 12 in]
  n170 = call <vilib>:"DAQmx Clear Task.vi"("task in"=w163, "error in"=w160) -> ("error out"=w50:errorcluster)  [unwired: 13 in]
  n171 = call <vilib>:"DAQmx Stop Task.vi"("task/channels in"=w47, "error in"=w50) -> ("task out"=w46:refnum<k21>, "error out"=w49:errorcluster)  [unwired: 12 in]
  n172 = call <vilib>:"DAQmx Clear Task.vi"("task in"=w46, "error in"=w49) -> ("error out"=w48:errorcluster)  [unwired: 13 in]
  n173 = Close File(refnum=w140, error in=w48) -> (error out=w132:errorcluster)  [unwired: 1 out]
  n174 = Close File(refnum=w139, error in=w132) -> (error out=w131:errorcluster)  [unwired: 1 out]
  n175 = Close File(refnum=w138, error in=w131) -> (error out=w63:errorcluster)  [unwired: 1 out]
  n176 = Close File(refnum=w64, error in=w63) -> (error out=w62:errorcluster)  [unwired: 1 out]
  n177 = call-poly <vilib>:"DAQmx Write.vi"("task/channels in"=w100, "data"=0.0, "error in"=w62) -> ("task out"=w99:refnum<k21>, "error out"=w97:errorcluster)  [unwired: 10 in, 1 out]
  n178 = call <vilib>:"DAQmx Stop Task.vi"("task/channels in"=w99, "error in"=w97) -> ("task out"=w98:refnum<k21>, "error out"=w96:errorcluster)  [unwired: 12 in]
  n179 = call <vilib>:"DAQmx Clear Task.vi"("task in"=w98, "error in"=w96) -> ("error out"=w30:errorcluster)  [unwired: 13 in]
  n180 = call <vilib>:"DAQmx Stop Task.vi"("task/channels in"=w80, "error in"=w30) -> ("task out"=w84:refnum<k21>, "error out"=w83:errorcluster)  [unwired: 12 in]
  n181 = call <vilib>:"DAQmx Clear Task.vi"("task in"=w84, "error in"=w83) -> ("error out"=w27:errorcluster)  [unwired: 13 in]
  n182 = call <vilib>:"DAQmx Stop Task.vi"("task/channels in"=w26, "error in"=w27) -> ("task out"=w29:refnum<k21>, "error out"=w28:errorcluster)  [unwired: 12 in]
  n183 = call <vilib>:"DAQmx Clear Task.vi"("task in"=w29, "error in"=w28) -> ("error out"=w4:errorcluster)  [unwired: 13 in]
  n184 = call <vilib>:"DAQmx Stop Task.vi"("task/channels in"=w2, "error in"=w4) -> ("task out"=w6:refnum<k21>, "error out"=w5:errorcluster)  [unwired: 12 in]
  n185 = call <vilib>:"DAQmx Clear Task.vi"("task in"=w6, "error in"=w5) -> ("error out"=w3:errorcluster)  [unwired: 13 in]
  n186 = call <vilib>:"Simple Error Handler.vi"("error in (no error)"=w3) -> ()  [unwired: 4 in, 5 out]
